vi "VIH - VI Doc Editor #2 - Get Non-terminal GenObject Refnums.vi"(8 "error in":errorcluster, 10 "Conpane Ctrl Refnums":refnum<vi>[](array[refnum]), 11 "VI Reference":refnum<vi>) -> (0 "error out":errorcluster, 2 "Non-terminal GenObject Refnums":refnum<vi>[](array[refnum]), 3 "dup VI Reference":refnum<vi>)   [LabVIEW 2014]
doc: "::: VI Helpeks :::\nCopyright (c) 2000-2026 Konstantin Shifershteyn. All rights reserved."
panel:
  # "VI Helpeks\nCopyright (c) 2012-2026 Konstantin Shifershteyn"
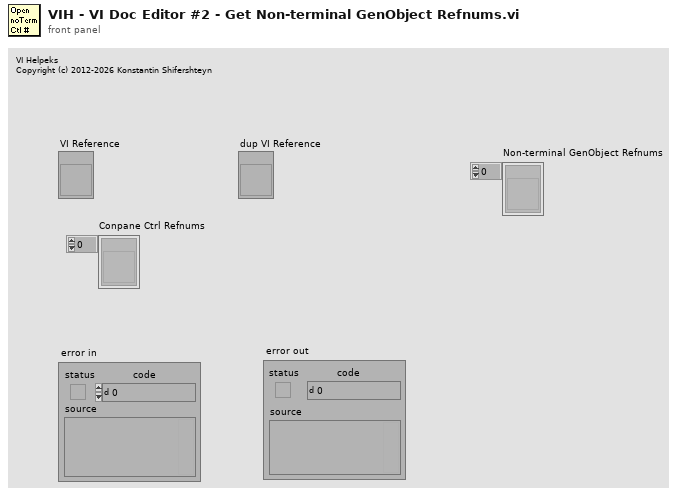
[diagram p1: front panel]
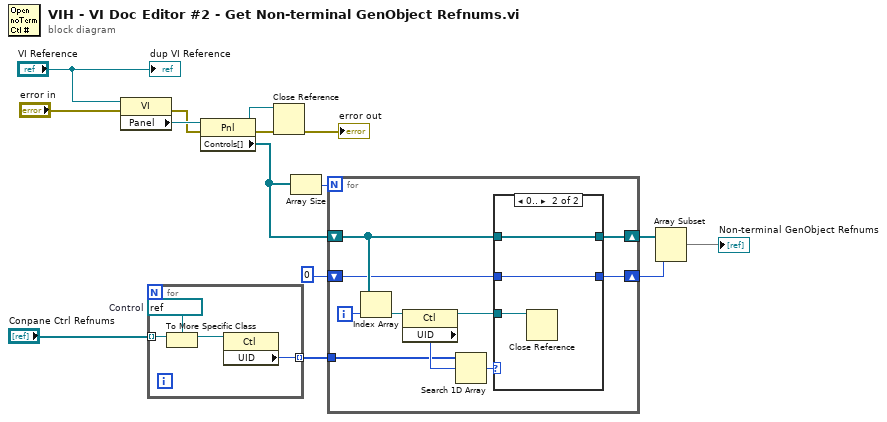
[diagram p0: block diagram]
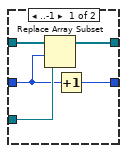
[diagram p2: hidden frame]
diagram:
  n1 = property class="VI"(reference="VI Reference", error in="error in") -> (error out=w13:errorcluster, "Panel"=w14:refnum<vi>)  [unwired: 1 out]
  n2 = for {
    tunnel: "Conpane Ctrl Refnums" -> [w19] mode=indexing
    tunnel: [w18] -> w7 mode=indexing
    w16 = refnum<vi> refnum  # Control
    n3 = To More Specific Class(target class=w16, reference=w19) -> (specific class reference=w17:refnum<vi>)  [unwired: 1 in, 1 out]
    n4 = property class="Ctl"(reference=w17) -> ("UID"=w18:i32)  [unwired: 1 in, 2 out]
  }
  n5 = property class="Pnl"(reference=w14, error in=w13) -> (reference out=w12:refnum<vi>, error out=w11:errorcluster, "Controls[]"=w6:refnum<vi>[])
  n6 = Close Reference(reference=w12, error in (no error)=w11) -> (error out=→"error out":errorcluster)
  n7 = Array Size(array=w6) -> (size(s)=w5:i32)
  n8 = for {
    N: w5 -> [_]
    tunnel: w7 -> [w28]
    shift-right: [w24] -> w3
    shift-left: w6 -> [w23]
    shift-right: [w21] -> w2
    shift-left: 0 -> [w20]
    i -> [w26]
    n9 = Index Array(array=w23, index=w26) -> (element=w27:refnum<vi>)
    n10 = property class="Ctl"(reference=w27) -> (reference out=w22:refnum<vi>, "UID"=w29:i32)  [unwired: 1 in, 1 out]
    n11 = Search 1D Array(1D array=w28, element=w29) -> (index of element=w25:i32)  [unwired: 1 in]
    n12 = case shown="0.." w25 {
      tunnel: [w33 w37] -> w24
      tunnel: w23 -> [w34 w37]
      tunnel: w22 -> [w32 w35]
      tunnel: [w30 w36] -> w21
      tunnel: w20 -> [w31 w36]
      frame ..-1 {
        n13 = Replace Array Subset(array=w34, new element=w32, index=w31) -> (w33:refnum<vi>[])
        n14 = Increment(x=w31) -> (x+1=w30:i32)
      }
      frame 0.. {
        n15 = Close Reference(reference=w35) -> ()  [unwired: 1 in, 1 out]
      }
    }
  }
  n16 = Array Subset(array=w3, length=w2) -> (→"Non-terminal GenObject Refnums":refnum<vi>[])  [unwired: 1 in]
  "dup VI Reference" <- "VI Reference"
